vi "C_Decode_WS_To_CAN.vi"(8 "error in (no error)":errorcluster, 9 "hdlc state in":T1, 10 "ws state in":T1, 11 "bytes in":u8[](array[numeric])) -> (0 "error out":errorcluster, 1 "hdlc state out":T1, 2 "ws state out":T1, 3 "frames":T3[](array[typedef]), 4 "ping payload":u8[](array[numeric]), 5 "result":T2)   [LabVIEW 2021, in "CANsub_C.lvlib"]
doc: "Decodes received TCP bytes (WebSocket + HDLC + CAN) into CAN frames. Incomplete data stays in the two states. result: frame count, peer close, ping length (-1 = none), CRC and decode errors. Allocates on every call: tests and setup; in the loop use C_Decode_RT."
uses:
  CANsub_C.lvlib
  common/Typedefs/Bytes.ctl
  common/CANsub_Common.lvlib
  common/Typedefs/CAN_Frame.ctl
  C_Decode_Result.ctl
  codec_vis/CANsub_Codec.lvlib
  C_State.ctl
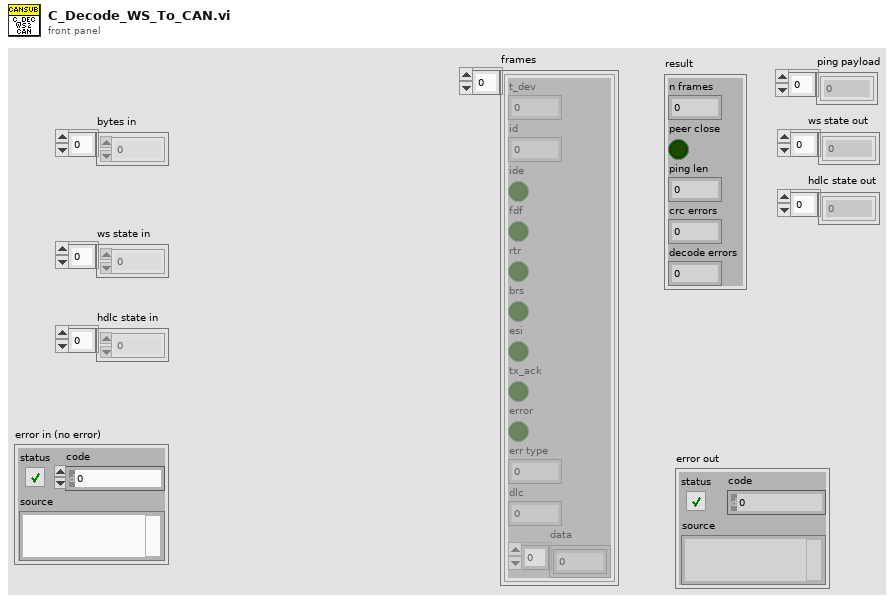
[diagram p1: front panel]
types:
  T1 = typedef "CANsub_C.lvlib/C_State.ctl" = u8[]
  T2 = typedef "CANsub_C.lvlib/C_Decode_Result.ctl" = cluster{"n frames":i32, "peer close":bool, "ping len":i32, "crc errors":u32, "decode errors":i32}
  T3 = typedef "CANsub_Common.lvlib/CAN_Frame.ctl" = cluster{"t_dev":dbl, "id":u32, "ide":bool, "fdf":bool, "rtr":bool, "brs":bool, "esi":bool, "tx_ack":bool, "error":bool, "err type":u8, "dlc":u8, "data":T4}
  T4 = typedef "CANsub_Common.lvlib/Bytes.ctl" = u8[]
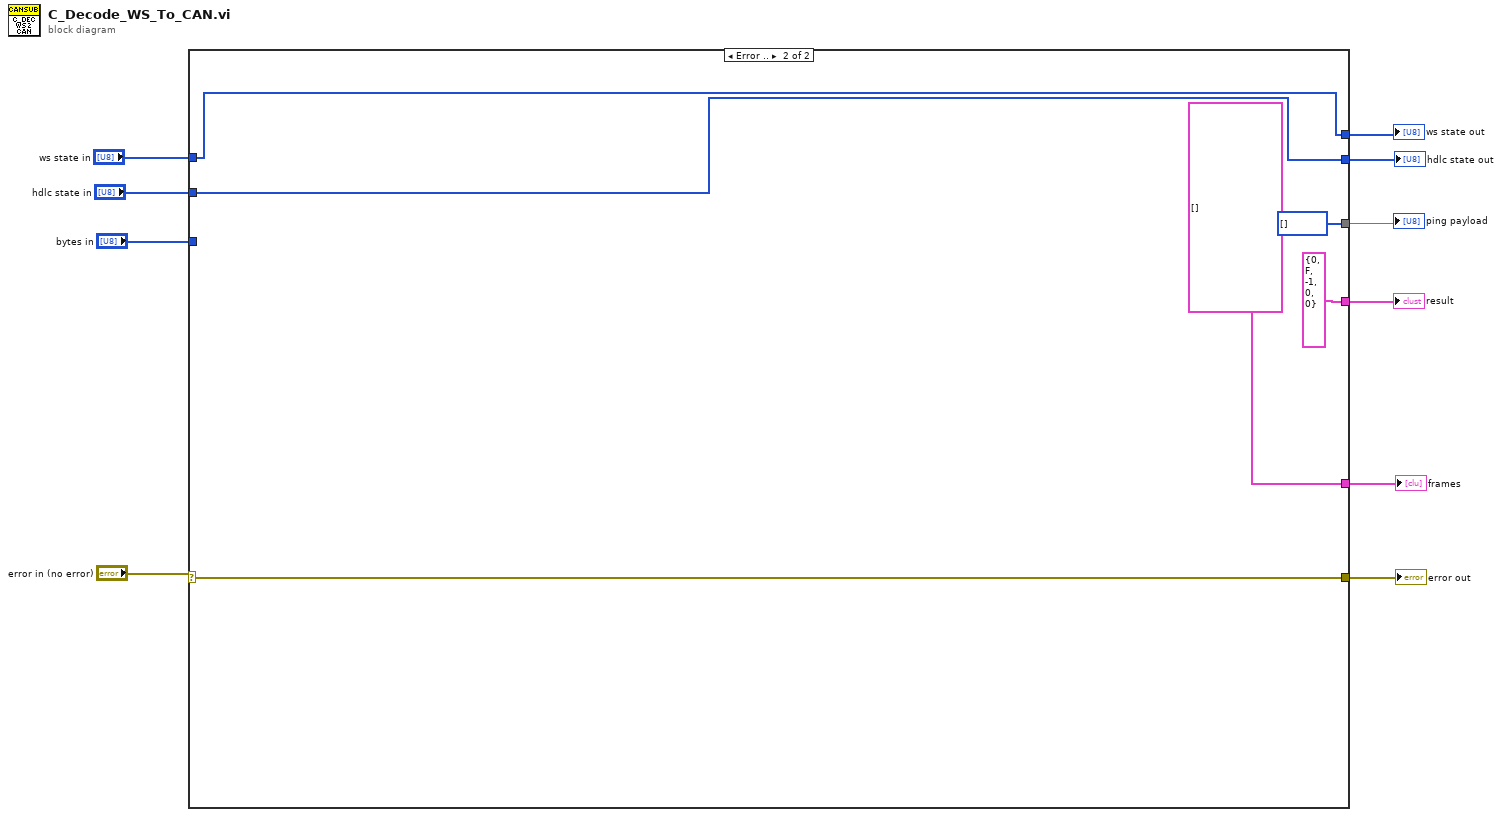
[diagram p0: block diagram]
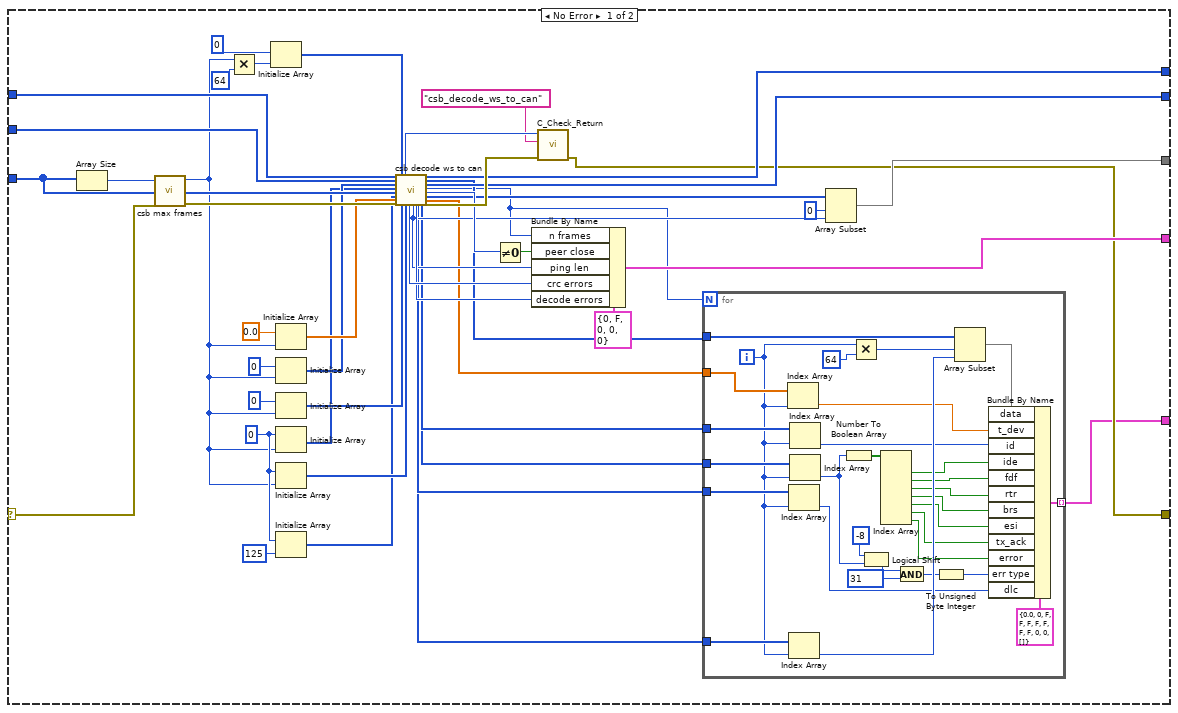
[diagram p2: hidden frame]
diagram:
  n1 = case shown="Error .." "error in (no error)" {
    selector: "error in (no error)" -> [w55 w92]
    tunnel: [w19 w92] -> w9
    tunnel: [w49 w91] -> w8
    tunnel: "ws state in" -> [w50 w91]
    tunnel: [w47 w90] -> w6
    tunnel: "hdlc state in" -> [w48 w90]
    tunnel: [w12 T3[] [] ("frames")] -> w4
    tunnel: [w20 u8[] [] ("ping payload")] -> w3
    tunnel: [w21 T2 {"n frames"=0, "peer close"=FALSE, "ping len"=-1, "crc errors"=0, "decode errors"=0} ("result")] -> w2
    tunnel: "bytes in" -> [w46 _]
    frame No Error {
      w45 = u8 0
      n2 = Array Size(array=w46) -> (size(s)=w56:i32)
      n3 = call "csb max frames.vi"("error in (no error)"=w55, "in_len"=w56) -> ("error out"=w52:errorcluster, "function return"=w41:i32)  [unwired: 8 in]
      n4 = Multiply(x=w41, y=64) -> (x*y=w39:i32)
      n5 = Initialize Array(u8 0, w39) -> (w32:u8[])
      n6 = Initialize Array(0.0, w41) -> (w37:dbl[])
      n7 = Initialize Array(u32 0, w41) -> (w36:u32[])
      n8 = Initialize Array(u16 0, w41) -> (w35:u16[])
      n9 = Initialize Array(w45, w41) -> (w34:u8[])
      n10 = Initialize Array(w45, w41) -> (w33:u8[])
      n11 = Initialize Array(w45, 125 ("dimension size")) -> (w31:u8[])
      n12 = call "csb decode ws to can.vi"("ws_state"=w50, "hdlc_state"=w48, "id"=w36, "dlc"=w34, "in"=w46, "ping_payload"=w31, "t_dev"=w37, "error in (no error)"=w52, "data"=w32, "flags"=w35, "data_len"=w33) -> ("function return"=w54:i32, "crc_errors"=w26:u32, "decode_errors"=w25:i32, "ping_len"=w22:i32, "dlc out"=w14:u8[], "data_len out"=w13:u8[], "id out"=w16:u32[], "flags out"=w15:u16[], "ws_state out"=w49:u8[], "data out"=w17:u8[], "hdlc_state out"=w47:u8[], "n_frames"=w11:i32, "peer_close"=w27:i32, "ping_payload out"=w24:u8[], "t_dev out"=w18:dbl[], "error out"=w51:errorcluster)  [unwired: 1 in]
      n13 = Not Equal To 0?(x=w27) -> (x != 0?=w28:bool)
      n14 = Bundle By Name(cluster=T2 {"n frames"=0, "peer close"=FALSE, "ping len"=0, "crc errors"=0, "decode errors"=0} ("C_Decode_Result"), "n frames"=w11, "peer close"=w28, "ping len"=w22, "crc errors"=w26, "decode errors"=w25) -> (w21:T2)
      n15 = call "C_Check_Return.vi"("error in (no error)"=w51, "function name"="csb_decode_ws_to_can", "function return"=w54) -> ("error out"=w19:errorcluster)  [unwired: 6 in, 2 out]
      n16 = for {
        N: w11 -> [_]
        tunnel: w17 -> [w86]
        tunnel: w18 -> [w85]
        tunnel: w16 -> [w84]
        tunnel: w15 -> [w83]
        tunnel: w14 -> [w82]
        tunnel: w13 -> [w81]
        tunnel: [w72] -> w12 mode=indexing
        i -> [w79]
        n17 = Index Array(array=w85, index=w79) -> (element=w74:dbl)
        n18 = Index Array(array=w82, index=w79) -> (element=w71:u8)
        n19 = Index Array(array=w81, index=w79) -> (element=w80:u8)
        n20 = Index Array(array=w84, index=w79) -> (element=w73:u32)
        n21 = Index Array(array=w83, index=w79) -> (element=w62:u16)
        n22 = Number To Boolean Array(number=w62) -> (Boolean array=w70:bool[])
        n23 = Multiply(x=w79, y=64) -> (x*y=w77:i32)
        n24 = Logical Shift(y=i16 -8, x=w62) -> (x << y=w60:u16)
        n25 = Index Array(array=w70) -> (element #1=w69:bool, element #2=w68:bool, element #3=w67:bool, element #4=w66:bool, element #5=w65:bool, element #6=w64:bool, element #7=w63:bool)  [unwired: 7 in]
        n26 = And(x=w60, y=u16 31) -> (x .and. y?=w58:u16)
        n27 = To Unsigned Byte Integer(number=w58) -> (unsigned 8bit integer=w57:u8)
        n28 = Array Subset(array=w86, index=w77, length=w80) -> (w75:u8[])
        n29 = Bundle By Name(cluster=T3 {"t_dev"=0.0, "id"=0, "ide"=FALSE, "fdf"=FALSE, "rtr"=FALSE, "brs"=FALSE, "esi"=FALSE, "tx_ack"=FALSE, "error"=FALSE, "err type"=0, "dlc"=0, "data"=[]} ("CAN_Frame"), "data"=w75, "t_dev"=w74, "id"=w73, "ide"=w69, "fdf"=w68, "rtr"=w67, "brs"=w66, "esi"=w65, "tx_ack"=w64, "error"=w63, "err type"=w57, "dlc"=w71) -> (w72:T3)
      }
      n30 = Array Subset(array=w24, index=0, length=w22) -> (w20:u8[])
    }
    frame Error {
    }
  }
  "frames" <- w4
  "result" <- w2
  "ws state out" <- w8
  "hdlc state out" <- w6
  "error out" <- w9
  "ping payload" <- w3
